vi "Input Parameter Cluster Label--constant.vi"() -> (3 "Input Parameter Cluster Label":string)   [LabVIEW 2026]
doc: "This constant defines the label of input parameter control (as a format string)."
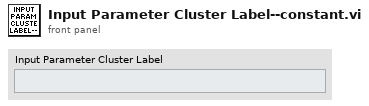
[diagram p1: front panel]
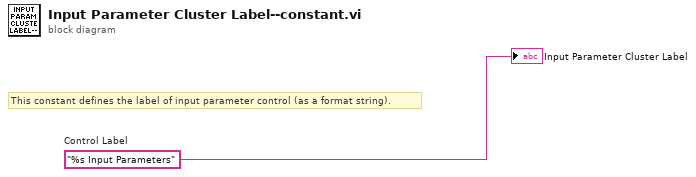
[diagram p0: block diagram]
diagram:
  w1 = "%s Input Parameters"  # Control Label
  # "This constant defines the label of input parameter control (as a format string)."
  "Input Parameter Cluster Label" <- w1
